vi "digital write.vi"(8 "error in (no error)":errorcluster, 9 "On/Off":bool, 10 "Line":string, 11 "USB-6001 in":refnum<class "USB-6001.lvclass">) -> (0 "error out":errorcluster, 3 "USB-6001 out":refnum<class "USB-6001.lvclass">)   [LabVIEW 2025, in "USB IO.lvlib" / "USB-6001.lvclass"]
uses:
  USB-6001.lvclass
  USB-6001.lvclass/USB-6001.ctl
  <vilib>/DAQmx/write.llb/DAQmx Write (Digital 1D Bool 1Chan 1Samp).vi
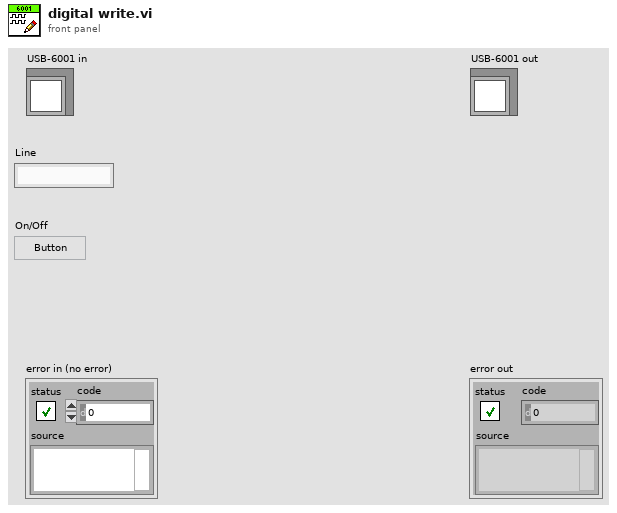
[diagram p1: front panel]
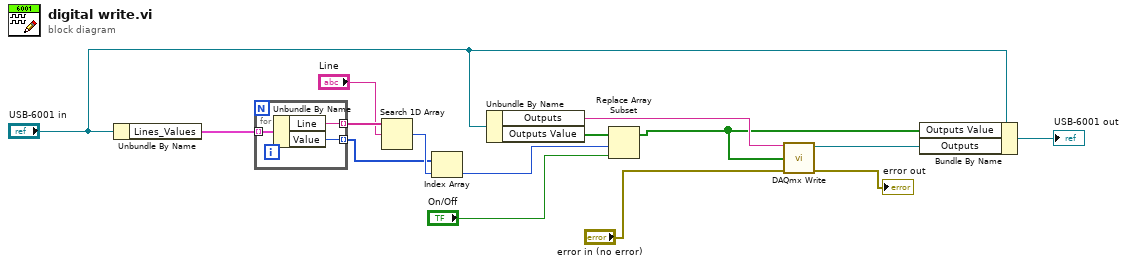
[diagram p0: block diagram]
diagram:
  n1 = Unbundle By Name("USB-6001 in") -> ("Lines_Values"=w15:cluster{"Line":string, "Value":i32}[])
  n2 = for {
    tunnel: w15 -> [w18] mode=indexing
    tunnel: [w17] -> w14 mode=indexing
    tunnel: [w16] -> w11 mode=indexing
    n3 = Unbundle By Name(w18) -> ("Line"=w17:string, "Value"=w16:i32)
  }
  n4 = Search 1D Array(1D array=w14, element="Line") -> (index of element=w12:i32)  [unwired: 1 in]
  n5 = Index Array(array=w11, index=w12) -> (element=w9:i32)
  n6 = Unbundle By Name("USB-6001 in") -> ("Outputs"=w5:string, "Outputs Value"=w10:bool[])
  n7 = Replace Array Subset(array=w10, new element="On/Off", index=w9) -> (w4:bool[])
  n8 = call-poly <vilib>:"DAQmx Write.vi"("task/channels in"=w5, "data"=w4, "error in"="error in (no error)") -> ("task out"=w1:refnum<k21>, "error out"=→"error out":errorcluster)  [unwired: 10 in, 1 out]
  n9 = Bundle By Name(cluster="USB-6001 in", "Outputs Value"=w4, "Outputs"=w1) -> (→"USB-6001 out":refnum<class "USB-6001.lvclass">)
